vi "ASK Demodulator.vi"(2 "Threshold":dbl, 3 "Samples per bit":i32, 4 "ASK Modulated Signal":dbl[](array[numeric])) -> (0 "Detected Energy":dbl[](array[numeric]), 1 "Recovered Binary Signal":i32[](array[numeric]))   [LabVIEW 2026]
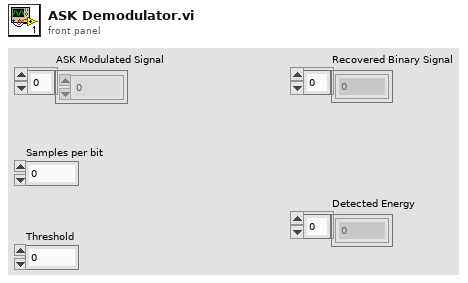
[diagram p1: front panel]
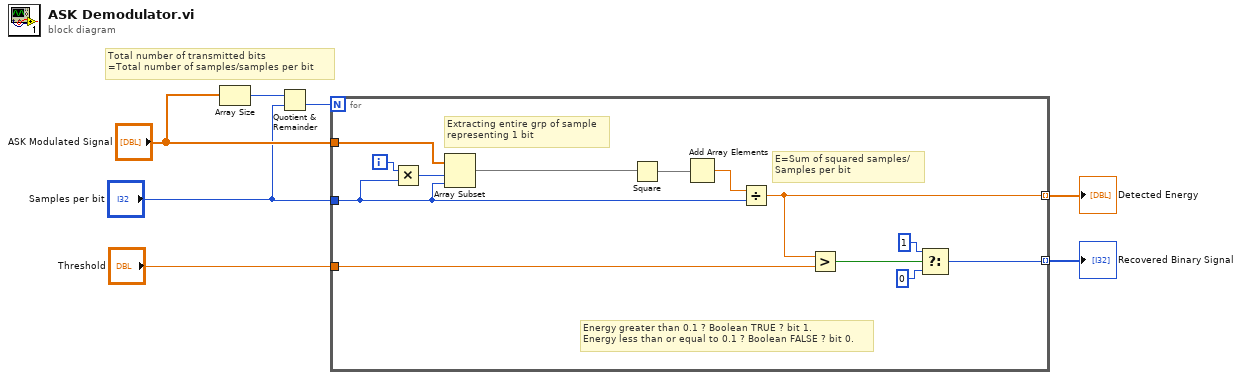
[diagram p0: block diagram]
diagram:
  # "Total number of transmitted bits\n=Total number of samples/samples per bit"
  n1 = Array Size(array="ASK Modulated Signal") -> (size(s)=w7:i32)
  n2 = Quotient & Remainder(x=w7, y="Samples per bit") -> (floor(x/y)=w6:i32)  [unwired: 1 out]
  n3 = for {
    N: w6 -> [_]
    tunnel: "ASK Modulated Signal" -> [w19]
    tunnel: "Samples per bit" -> [w14]
    tunnel: [w13] -> w3 mode=indexing
    tunnel: "Threshold" -> [w12]
    tunnel: [w8] -> w1 mode=indexing
    i -> [w20]
    # "Energy greater than 0.1 ? Boolean TRUE ? bit 1.\nEnergy less than or equal to 0.1 ? Boolean FALSE ? bit 0."
    # "E=Sum of squared samples/\nSamples per bit"
    # "Extracting entire grp of sample\nrepresenting 1 bit"
    n4 = Multiply(x=w20, y=w14) -> (x*y=w18:i32)
    n5 = Array Subset(array=w19, index=w18, length=w14) -> (w17:dbl[])
    n6 = Square(x=w17) -> (x^2=w16:dbl[])
    n7 = Add Array Elements(numeric array=w16) -> (sum=w15:dbl)
    n8 = Divide(x=w15, y=w14) -> (x/y=w13:dbl)
    n9 = Greater?(x=w13, y=w12) -> (0:w11:bool)
    n10 = Select(t=1, s=w11, f=0) -> (s? t:f=w8:i32)
  }
  "Recovered Binary Signal" <- w1
  "Detected Energy" <- w3
